vi "Dirty Probe.vi"(0 "vi path":string) -> (4 "vi mods":i32, 6 "bd mods":i32, 8 "fp mods":i32, 10 "user changes":bool, 15 "error out":errorcluster)   [LabVIEW 2026]
doc: "Open a VI by path and report its modification state. Reads the VI, block diagram and front panel modification bitsets and the User Changes flag over VI Server, then releases the reference. Used to test whether a VI that was patched on disk still loads clean."
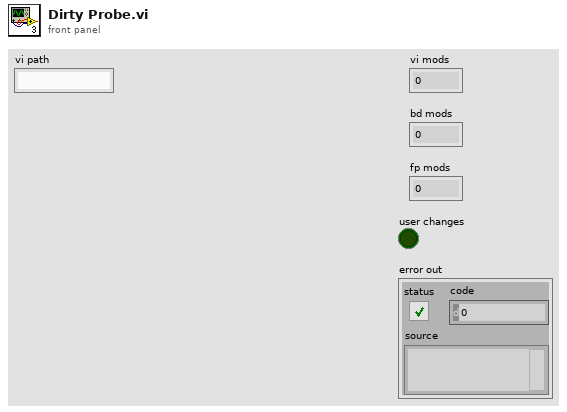
[diagram p1: front panel]
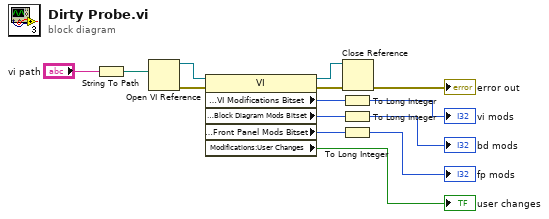
[diagram p0: block diagram]
diagram:
  n1 = String To Path(string="vi path") -> (path=w13:path)
  n2 = Open VI Reference(vi path=w13) -> (vi reference=w12:refnum<vi>, error out=w11:errorcluster)  [unwired: 5 in]
  n3 = property class="VI"(reference=w12, error in=w11) -> (reference out=w3:refnum<vi>, error out=w2:errorcluster, "Modifications:VI Modifications Bitset"=w10:u64, "Modifications:Block Diagram Mods Bitset"=w9:u32, "Modifications:Front Panel Mods Bitset"=w8:u32, "Modifications:User Changes"=→"user changes":bool)
  n4 = To Long Integer(number=w10) -> (32bit integer=→"vi mods":i32)
  n5 = To Long Integer(number=w9) -> (32bit integer=→"bd mods":i32)
  n6 = To Long Integer(number=w8) -> (32bit integer=→"fp mods":i32)
  n7 = Close Reference(reference=w3, error in (no error)=w2) -> (error out=→"error out":errorcluster)
